vi "Transport_Close.vi"(8 "error in (no error)":errorcluster={"status"=FALSE, "code"=0, "source"="\"\""}, 11 "Channel references":string) -> (0 "error out":errorcluster={"status"=FALSE, "code"=0, "source"="\"\""}, 2 "status ok":bool, 3 "Final status":string)   [LabVIEW 2026]
doc: "INTENT: Release endpoints. LOGIC: Signal close, release endpoints and flush bounded essential messages where possible."
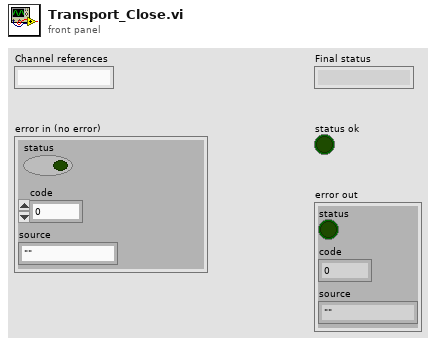
[diagram p1: front panel]
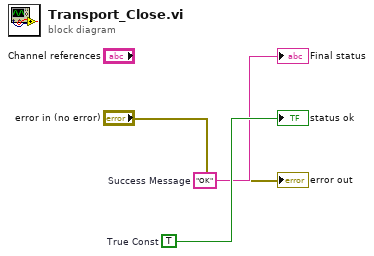
[diagram p0: block diagram]
diagram:
  w3 = TRUE  # True Const
  w2 = "OK"  # Success Message
  "Final status" <- w2
  "status ok" <- w3
  "error out" <- "error in (no error)"
